vi "Set Python Module.vi"(8 "error in":errorcluster, 10 "Python Module":path, 11 "Runner in":refnum<class "Runner.lvclass">) -> (0 "error out":errorcluster, 3 "Runner out":refnum<class "Runner.lvclass">)   [LabVIEW 2026, in "Runner.lvlib" / "Runner.lvclass"]
doc: "Set Python Module."
uses:
  Runner.lvclass
  Runner.lvclass/Runner.ctl
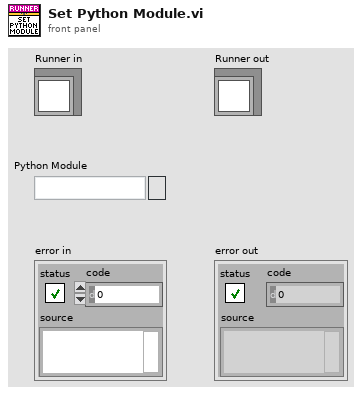
[diagram p1: front panel]
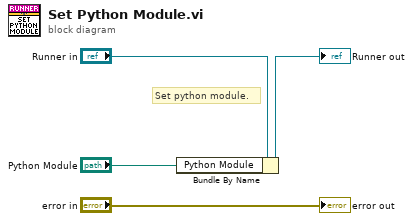
[diagram p0: block diagram]
diagram:
  # "Set python module."
  n1 = Bundle By Name(cluster="Runner in", "Python Module"="Python Module") -> (→"Runner out":refnum<class "Runner.lvclass">)
  "error out" <- "error in"
